vi "00 - Calling Python Simple.vi"() -> ()   [LabVIEW 2026]
panel:
  out "Intensity Graph":dbl[][](graph)
  in  "Colormap to Extract":string="viridis"
  out "return value":cluster{"R":dbl, "G":dbl, "B":dbl, "A":dbl}[](array[cluster])
  out "Colormap Names":string[](array[string])
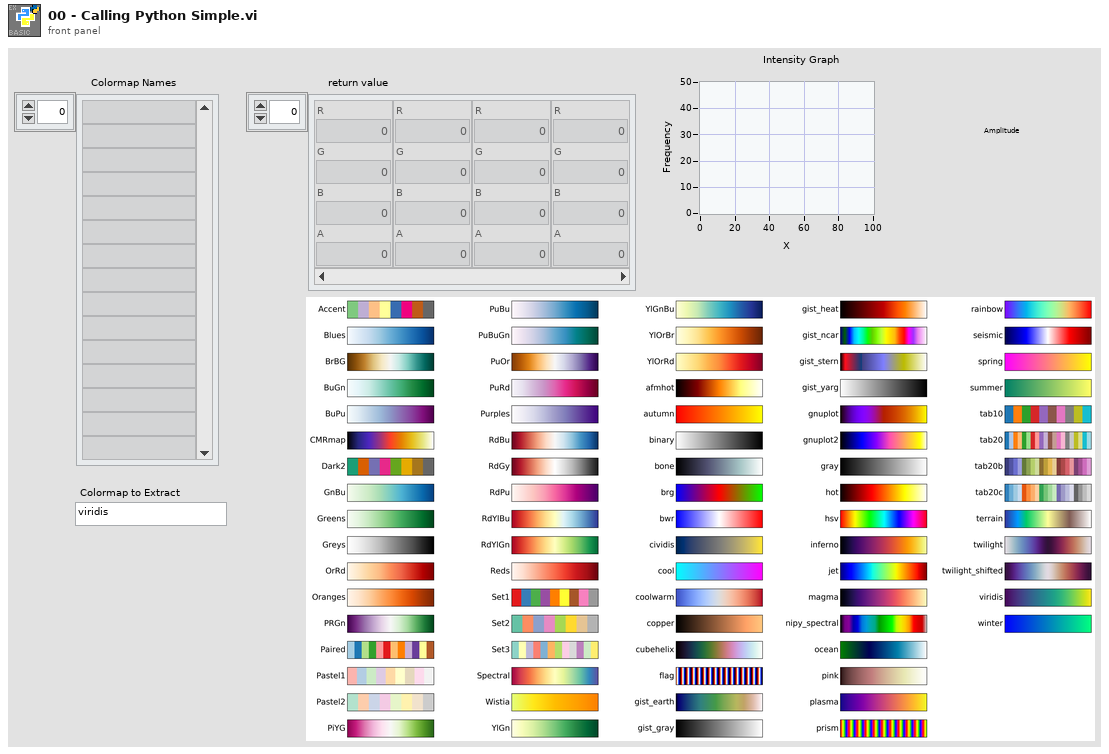
[diagram p1: front panel]
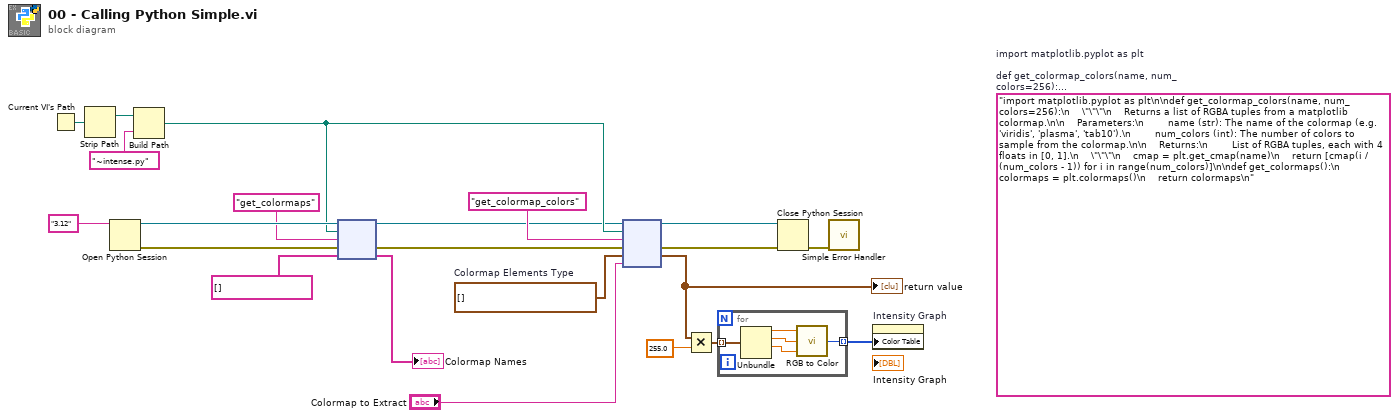
[diagram p0: block diagram]
diagram:
  w22 = cluster{"R":dbl, "G":dbl, "B":dbl, "A":dbl}[] []  # Colormap Elements Type
  (unwired) "import matplotlib.pyplot as plt\n\ndef get_colormap_colors(name, num_colors=256):\n    \"\"\"\n    Returns a list of RGBA tuples from a matplotlib colormap.\n\n    Parameters:\n        name (str): The name of the colormap (e.g. 'viridis', 'plasma', 'tab10').\n        num_colors (int): The number of colors to sample from the colormap.\n\n    Returns:\n        List of RGBA tuples, each with 4 floats in [0, 1].\n    \"\"\"\n    cmap = plt.get_cmap(name)\n    return [cmap(i / (num_colors - 1)) for i in range(num_colors)]\n\ndef get_colormaps():\n    colormaps = plt.colormaps()\n    return colormaps\n"  # import matplotlib.pyplot as plt  def get_colormap_colors(name, num_colors=256):     """     Returns a list of RGBA tuples from a matplotlib colormap.      Parameters:         name (str): The name of the colormap (e.g. 'viridis', 'plasma', 'tab10').         num_colors (int): The number of colors to sample from the colormap.      Returns:         List of RGBA tuples, each with 4 floats in [0, 1].     """     cmap = plt.get_cmap(name)     return [cmap(i / (num_colors - 1)) for i in range(num_colors)]  def get_colormaps():     colormaps = plt.colormaps()     return colormaps
  n1 = Current VI's Path() -> (path=w13:path)
  n2 = Strip Path(path=w13) -> (stripped path=w14:path)  [unwired: 1 out]
  n3 = Open Python Session(python version="3.12" ("Python version")) -> (session out=w20:refnum<k35>, error out=w21:errorcluster)  [unwired: 2 in]
  n4 = Build Path(base path=w14, name or relative path="~intense.py" ("function name")) -> (appended path=w10:path)
  n5 = node(w20, w10, "get_colormaps" ("function name"), w21, string[] [] ("function name")) -> (w9:refnum<k35>, w8:errorcluster, →"Colormap Names":string[])  [unwired: 2 out]
  n6 = node(w9, w10, "get_colormap_colors" ("function name"), w8, w22, "Colormap to Extract") -> (w6:refnum<k35>, w7:errorcluster, w4:cluster{"R":dbl, "G":dbl, "B":dbl, "A":dbl}[])  [unwired: 1 in, 2 out]
  "return value" <- w4
  n7 = Multiply(x=w4, y=255.0 ("A")) -> (x*y=w3:cluster{"R":dbl, "G":dbl, "B":dbl, "A":dbl}[])
  n8 = for {
    tunnel: w3 -> [w27] mode=indexing
    tunnel: [w23] -> w1 mode=indexing
    n9 = Unbundle(w27) -> ("R"=w26:dbl, "G"=w25:dbl, "B"=w24:dbl)  [unwired: 1 out]
    n10 = call <vilib>:"RGB to Color.vi"("B"=w24, "G"=w25, "R"=w26) -> ("Color"=w23:u32)
  }
  n11 = Close Python Session(session in=w6, error in=w7) -> (11:w15:errorcluster)
  n12 = call <vilib>:"Simple Error Handler.vi"("error in (no error)"=w15) -> ()  [unwired: 4 in, 5 out]
  n13 = property on="Intensity Graph" class="IntGraph (strict)"("Color Table"=w1) -> ()  [unwired: 2 in, 2 out]
